vi "GpuMat Clone.vi"(8 "error in (no error)":errorcluster, 11 "Src in":refnum<class "GpuMat.lvclass">) -> (0 "error out":errorcluster, 2 "Clone out":refnum<class "GpuMat.lvclass">, 3 "Src out":refnum<class "GpuMat.lvclass">)   [LabVIEW 2020, in "OpenLvVision_OpenCv.lvlib" / "Cuda.lvlib" / "GpuMat.lvclass"]
doc: "Returns deep copy of the matrix, i.e. the data is copied"
uses:
  GpuMat.lvclass
  OpenLvVision_OpenCv.lvlib
  <vilib>/Utility/error.llb/Error Cluster From Error Code.vi
  <vilib>/ErrorRing/Error Ring.xnode
  _LvHelpers/EdvrObject/EdvrObject.lvclass
  _LvHelpers/EdvrObject/TypeDef/Edvr.ctl
  Dlls/OlvOpenCvWrapper.dll
  C:/Users/lukas/Documents/OpenLvVision_OpenCv/SourceCode/LabView/OpenLvVision_OpenCv/_LvHelpers/EdvrObject/EdvrObject.lvclass
  C:/Users/lukas/Documents/OpenLvVision_OpenCv/SourceCode/LabView/OpenLvVision_OpenCv/Cuda/DataAccess/GpuMat/GpuMat.lvclass
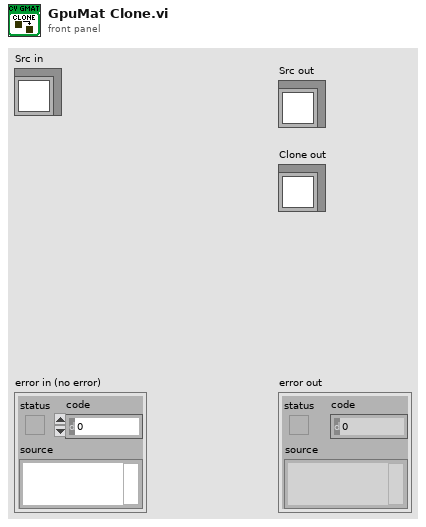
[diagram p1: front panel]
types:
  T1 = typedef "OpenLvVision_OpenCv.lvlib/EdvrObject.lvclass/Edvr.ctl" = refnum<data-value>
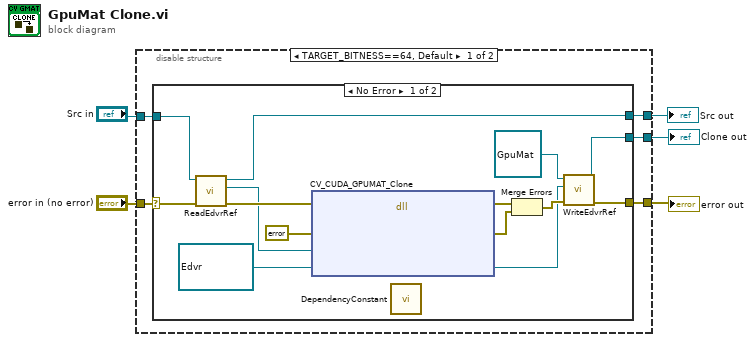
[diagram p0: block diagram]
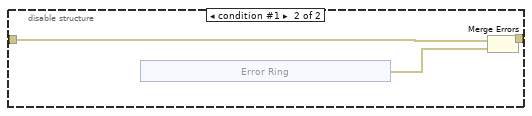
[diagram p3: hidden frame]
diagram:
  n1 = disable-structure shown="TARGET_BITNESS==64, Default" {
    disable-tunnel: "error in (no error)" -> [w10 w28]
    disable-tunnel: [w9 w29] -> w5
    disable-tunnel: "Src in" -> [w8 _]
    disable-tunnel: [w7 _] -> w2
    disable-tunnel: [w6 _] -> w1
    frame condition #0 (active) {
      n2 = case shown="No Error" w10 {
        selector: w10 -> [w17 w26]
        tunnel: [w15 w26] -> w9
        tunnel: w8 -> [w19 w25]
        tunnel: [w18 w25] -> w7
        tunnel: [w13 _] -> w6
        frame No Error {
          n3 = call "ReadEdvrRef.vi"("error in (no error)"=w17, "EdvrObject in"=w19) -> ("error out"=w21:errorcluster, "Edvr"=w20:T1, "EdvrObject out"=w18:refnum<class "GpuMat.lvclass">)  [unwired: 7 in]
          n4 = dll-call lib="C:/Users/lukas/Documents/OpenLvVision_OpenCv/SourceCode/LabView/OpenLvVision_OpenCv/Dlls/OlvOpenCvWrapper.dll" fn="CV_CUDA_GPUMAT_Clone"(error in=w21, "Error"=errorcluster {"status"=FALSE, "code"=0, "source"=""} ("error out"), "srcRef"=w20, "dstRef"=T1 refnum ("Edvr")) -> (error out=w24:errorcluster, "Error"=w23:errorcluster, "dstRef"=w12:T1)  [unwired: 4 in, 1 out]
          n5 = call "DependencyConstant.vi"() -> ()  [unwired: 12 in]
          n6 = Merge Errors(w24, w23) -> (w16:errorcluster)
          n7 = call "WriteEdvrRef.vi"("error in (no error)"=w16, "Edvr"=w12, "EdvrObject in"=refnum<class "GpuMat.lvclass"> refnum ("Dst out")) -> ("error out"=w15:errorcluster, "EdvrObject out"=w13:refnum<class "GpuMat.lvclass">)  [unwired: 7 in]
        }
        frame Error {
        }
      }
    }
    frame condition #1 {
      n8 = xnode "Error Ring"() -> ("error out"=w27:errorcluster)
      n9 = Merge Errors(w28, w27) -> (w29:errorcluster)
    }
  }
  "error out" <- w5
  "Clone out" <- w1
  "Src out" <- w2
